vi "all select for seqlist.vi"(7 "path":string="000.csv", 9 "Cluster":T4={"Right Read MIN"=6, "STD Type"=enum."Region", "Selection"=enum."10kHz", "Filter P"=0, "noise MAX"=3}, 10 "sample name":string[](array[string]), 11 "Seq":string[](array[string])) -> (3 "S array":T1(array[cluster]))   [LabVIEW 2018]
panel:
  out "S New Info and MiN out":T2={"Sample Sequence"="GATGATGATGATGATGAT", "Right Read MIN"=6, "Filter P"=0, "STD Type"=enum."Region", "Base Table"=[], "Selection"=enum."10kHz", "noise MAX"=3, "Sample name"=""} {"Base Table"."Value 3" format="%.2g"}
  out "Base Table":T3(array[cluster]) {"Value 3" format="%.2g"}
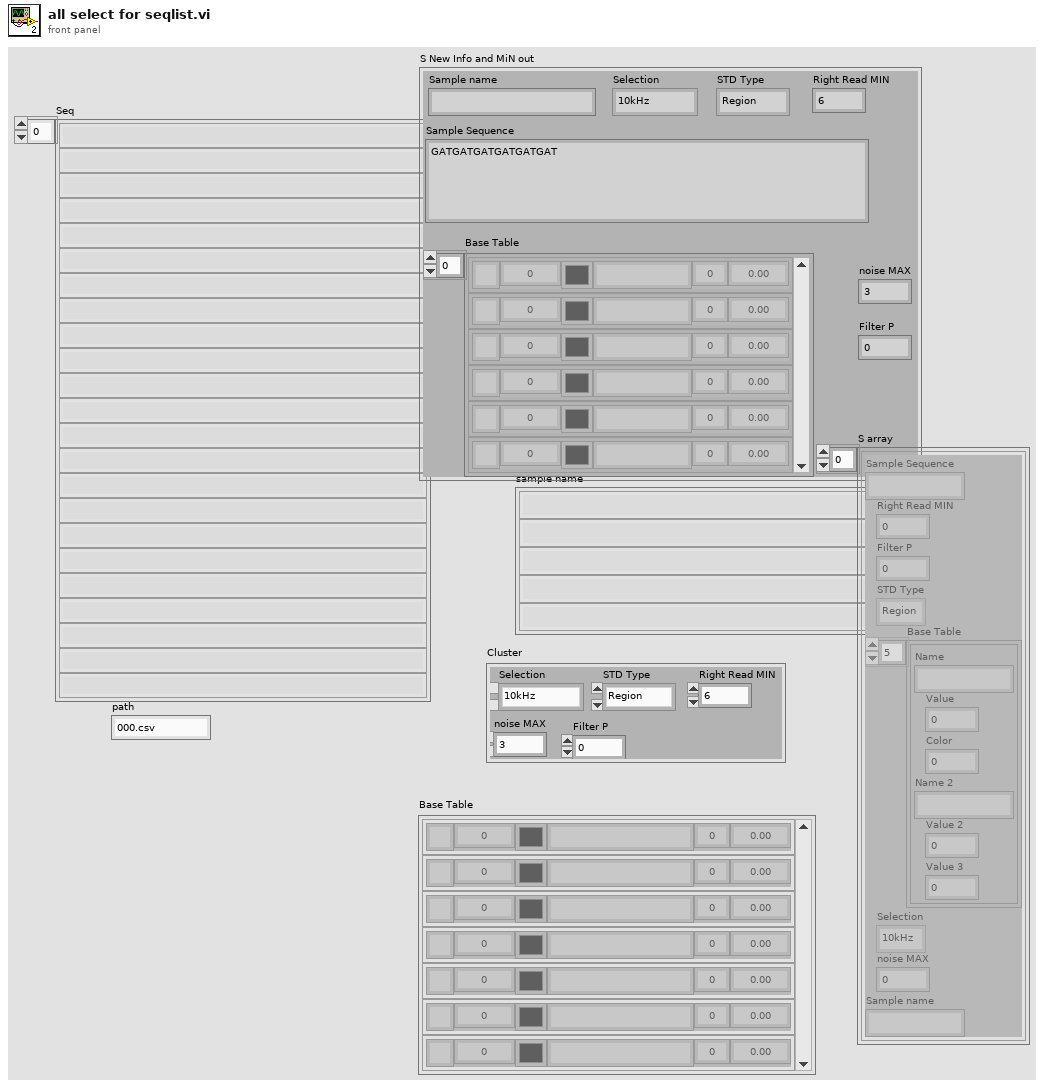
[diagram p1: front panel]
types:
  T1 = cluster{"Sample Sequence":string, "Right Read MIN":i32, "Filter P":i32, "STD Type":enum16{"Region", "Each", "Fixed"}, "Base Table":cluster{"Name":string, "Value":dbl, "Color":u32, "Name 2":string, "Value 2":dbl, "Value 3":dbl}[], "Selection":enum16{"10kHz", "100kHz"}, "noise MAX":i32, "Sample name":string}[]
  T2 = cluster{"Sample Sequence":string, "Right Read MIN":i32, "Filter P":i32, "STD Type":enum16{"Region", "Each", "Fixed"}, "Base Table":cluster{"Name":string, "Value":dbl, "Color":u32, "Name 2":string, "Value 2":dbl, "Value 3":dbl}[], "Selection":enum16{"10kHz", "100kHz"}, "noise MAX":i32, "Sample name":string}
  T3 = cluster{"Name":string, "Value":dbl, "Color":u32, "Name 2":string, "Value 2":dbl, "Value 3":dbl}[]
  T4 = cluster{"Right Read MIN":i32, "STD Type":enum16{"Region", "Each", "Fixed"}, "Selection":enum16{"10kHz", "100kHz"}, "Filter P":i32, "noise MAX":i32}
  T5 = cluster{"Sample ID":string, "Right Read MIN":i32, "Filter P":i32, "STD Type":enum16{"Region", "Each", "Fixed"}, "Base All Composition":cluster{"Name":string, "Value":dbl, "Color":u32, "Name 2":string, "Value 2":dbl, "Value 3":dbl}[], "Selection":enum16{"10kHz", "100kHz"}, "noise MAX":i32, string}
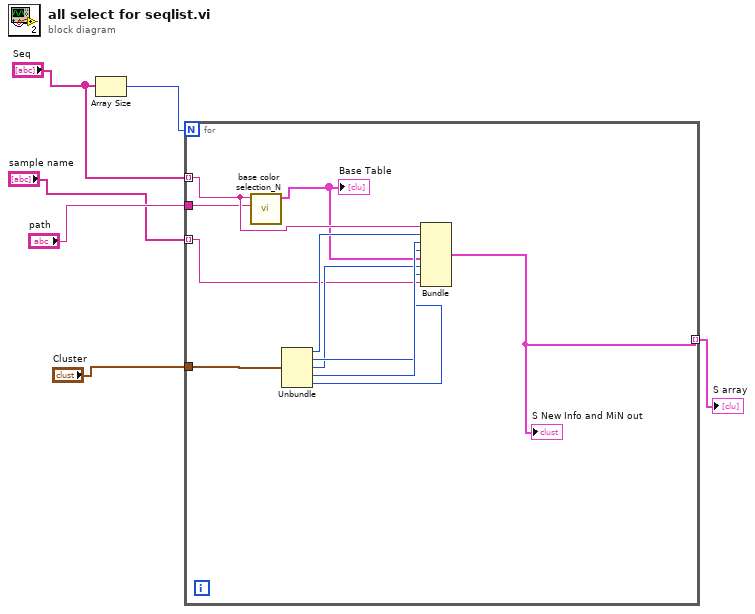
[diagram p0: block diagram]
diagram:
  n1 = Array Size(array="Seq") -> (size(s)=w6:i32)
  n2 = for {
    N: w6 -> [_]
    tunnel: "Seq" -> [w15] mode=indexing
    tunnel: "sample name" -> [w9] mode=indexing
    tunnel: "Cluster" -> [w17]
    tunnel: [w8] -> w4 mode=indexing
    tunnel: "path" -> [w7]
    n3 = call "base color selection_N.vi"("path"=w7, "Sample Sequence"=w15) -> ("Base All Composition"=w12:T3)  [unwired: 8 in, 1 out]
    "Base Table" <- w12
    n4 = Unbundle(w17) -> ("Right Read MIN"=w16:i32, "STD Type"=w13:enum16{"Region", "Each", "Fixed"}, "Selection"=w11:enum16{"10kHz", "100kHz"}, "Filter P"=w14:i32, "noise MAX"=w10:i32)
    n5 = Bundle("Sample ID"=w15, "Right Read MIN"=w16, "Filter P"=w14, "STD Type"=w13, "Base All Composition"=w12, "Selection"=w11, "noise MAX"=w10, w9) -> (w8:T5)  [unwired: 1 in]
    "S New Info and MiN out" <- w8
  }
  "S array" <- w4
